vi "Build CE Deploy - Check Path for Exclusion.vi"(8 "Exclude folder names":string[](array[string]), 9 "Exclude file name patterns":string[](array[string]), 10 "Path":path, 11 "Base dir":path) -> (2 "pass":bool)   [LabVIEW 2021]
doc: "::: CalcExpress Toolkit :::\nCopyright (c) 2000-2026 Konstantin Shifershteyn. All rights reserved."
panel:
  # "CalcExpress Toolkit\nCopyright (c) 2000-2026 Konstantin Shifershteyn"
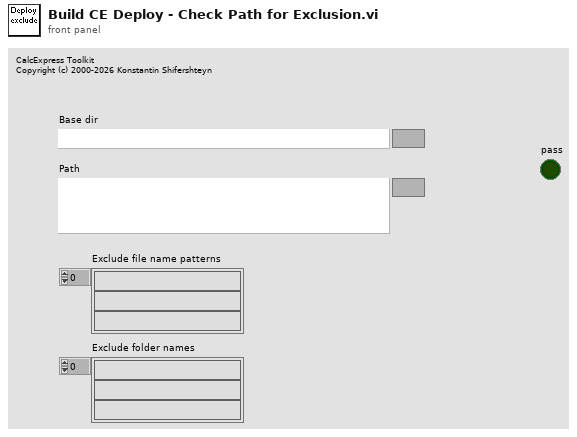
[diagram p1: front panel]
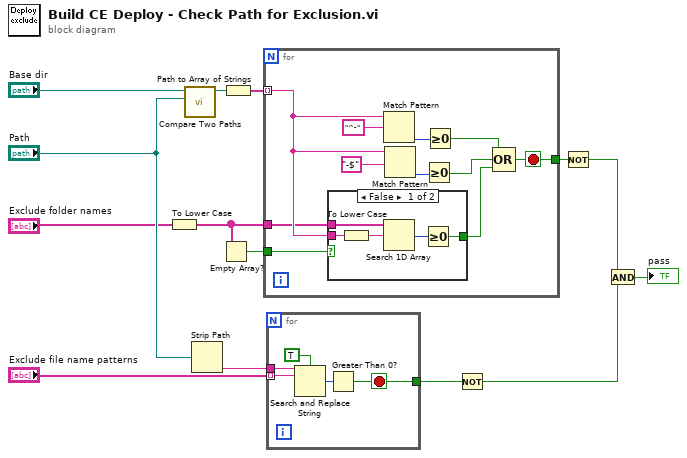
[diagram p0: block diagram]
diagram:
  n1 = To Lower Case(string="Exclude folder names") -> (all lower case string=w5:string[])
  n2 = call <vilib>:"Compare Two Paths.vi"("Path 2"="Path", "Path 1"="Base dir") -> ("Relative Path from 1 to 2"=w13:path)  [unwired: 6 in, 3 out]
  n3 = Strip Path(path="Path") -> (name=w9:string)  [unwired: 1 out]
  n4 = Empty Array?(array=w5) -> (empty?=w10:bool)
  n5 = Path to Array of Strings(0:w13) -> (2:w12:string[])  [unwired: 1 out]
  n6 = for {
    tunnel: w12 -> [w18] mode=indexing
    tunnel: [w19] -> w11
    tunnel: w5 -> [w17]
    tunnel: w10 -> [w15]
    stop <- w19 stop-if-true
    n7 = case shown="False" w15 {
      tunnel: w18 -> [w30 _]
      tunnel: w17 -> [w29 _]
      tunnel: [w26 _] -> w16
      frame False {
        n8 = To Lower Case(string=w30) -> (all lower case string=w28:string)
        n9 = Search 1D Array(1D array=w29, element=w28) -> (index of element=w27:i32)  [unwired: 1 in]
        n10 = Greater Or Equal To 0?(x=w27) -> (x >= 0?=w26:bool)
      }
      frame True {
      }
    }
    n11 = Match Pattern(string=w18, regular expression="^-") -> (offset past match=w24:i32)  [unwired: 1 in, 3 out]
    n12 = Match Pattern(string=w18, regular expression="-$") -> (offset past match=w25:i32)  [unwired: 1 in, 3 out]
    n13 = Greater Or Equal To 0?(x=w25) -> (x >= 0?=w20:bool)
    n14 = Greater Or Equal To 0?(x=w24) -> (x >= 0?=w21:bool)
    n15 = Compound Arithmetic op=OR(w21, w20, w16) -> (w19:bool)
  }
  n16 = for {
    tunnel: "Exclude file name patterns" -> [w34] mode=indexing
    tunnel: w9 -> [w35]
    tunnel: [w31] -> w7
    stop <- w31 stop-if-true
    n17 = Search and Replace String(case sensitive?=TRUE, input string=w35, search string=w34) -> (number of replacements=w32:i32)  [unwired: 5 in, 3 out]
    n18 = Greater Than 0?(x=w32) -> (x > 0?=w31:bool)
  }
  n19 = Not(x=w7) -> (.not. x?=w2:bool)
  n20 = Not(x=w11) -> (.not. x?=w3:bool)
  n21 = And(x=w3, y=w2) -> (x .and. y?=→"pass":bool)
